vi "ATM Scaffold.vi"() -> ()   [LabVIEW 2026]
doc: "ATM controller for the CLD ATM exam, built on the Bank DQMH module. An event loop (producer) turns every front panel action into a command string on a queue - Insert Card, Terminate, Enter=<User Input>, the action of a pressed menu button, or Activity for a keystroke - so the value the consumer needs travels with the command. A command loop (consumer) dequeues them and runs the state machine in Handle ATM Command.vi, which asks the Bank module for every account operation; the GUI never touches the accounts file. Apply ATM UI State.vi then enables, disables, focuses and fills the panel for the new mode. A dequeue timeout of 10 s after card insertion is the inactivity timer, and every keystroke in User Input re-arms it. Return Card, the timeout and an error release Card Simulator with a signalling write, which ends the event loop and, through Terminate, the command loop. Shut Down ATM.vi then releases the queue, closes the panel reference and stops the Bank module."
panel:
  out "Right Menu":T1
  out "Left Menu":T1
  out "ATM Messages":string
  in  "Right Buttons":T2
  in  "Left Buttons":T2
  in  "User Input":string
  in  "Enter":bool
  in  "Card Simulator":bool
  out "error out":errorcluster
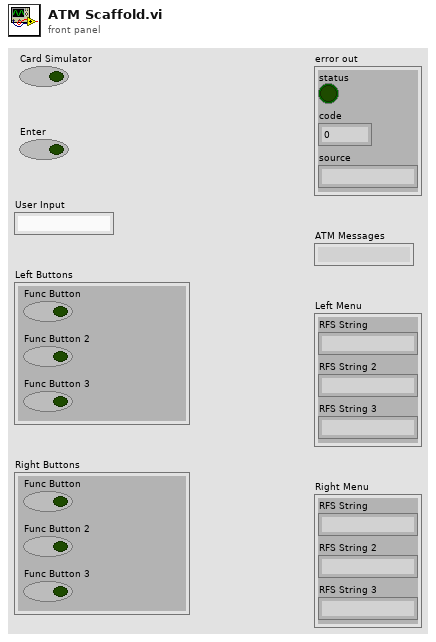
[diagram p1: front panel]
types:
  T1 = cluster{"RFS String":string, "RFS String 2":string, "RFS String 3":string}
  T2 = cluster{"Func Button":bool, "Func Button 2":bool, "Func Button 3":bool}
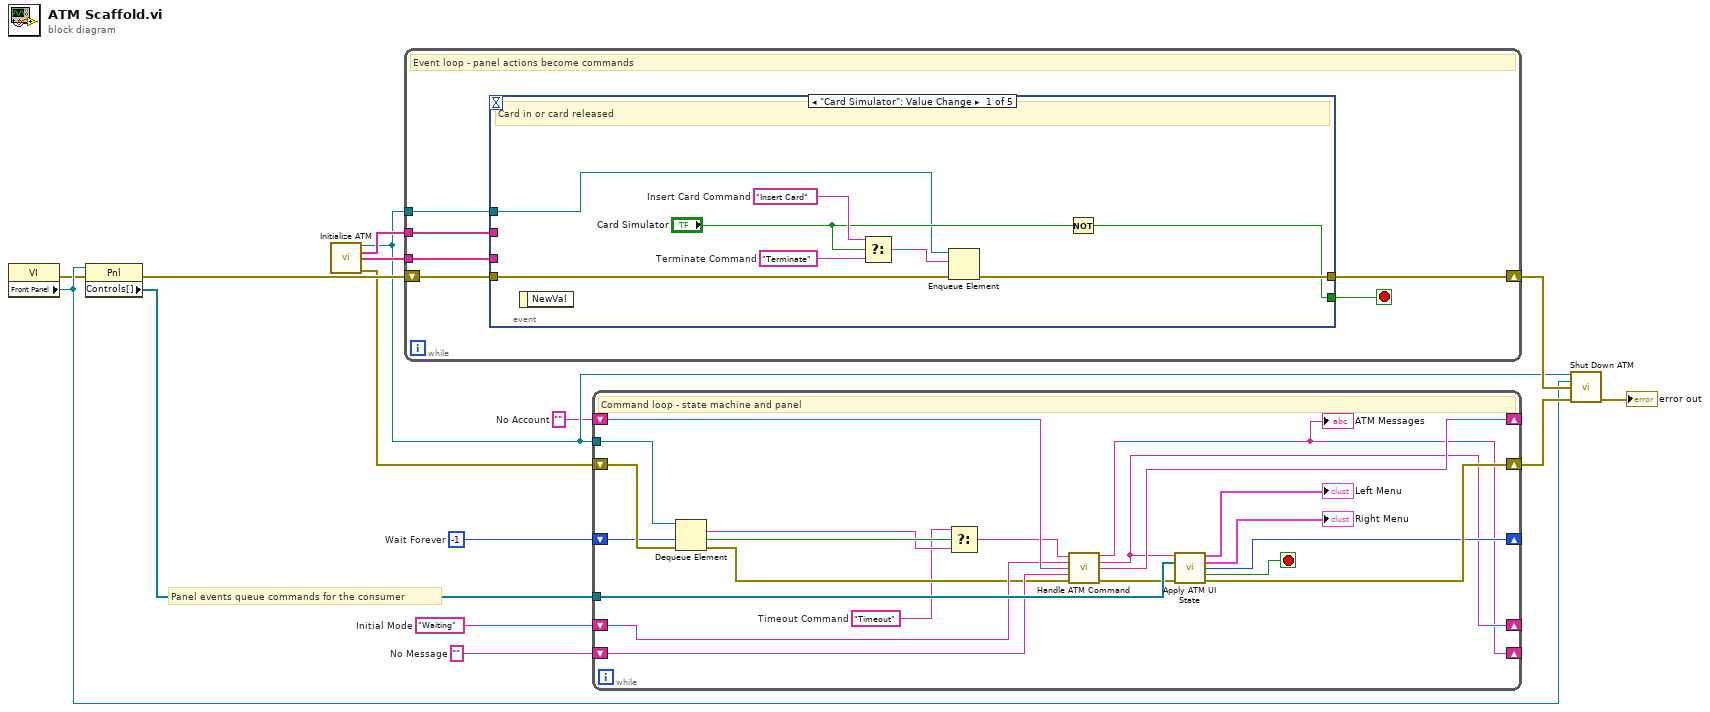
[diagram p0: block diagram]
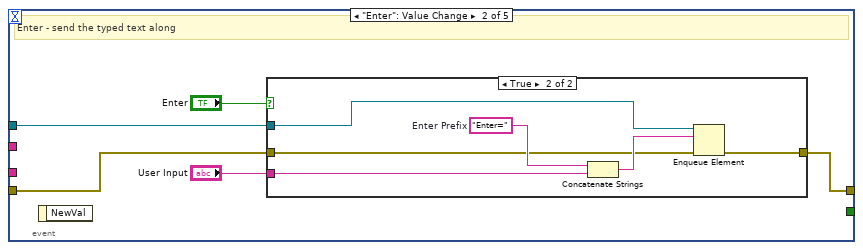
[diagram p2: hidden frame]
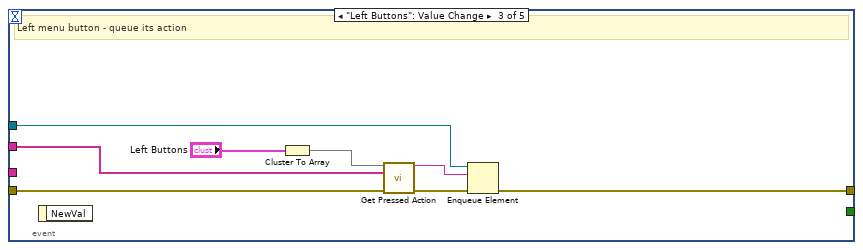
[diagram p4: hidden frame]
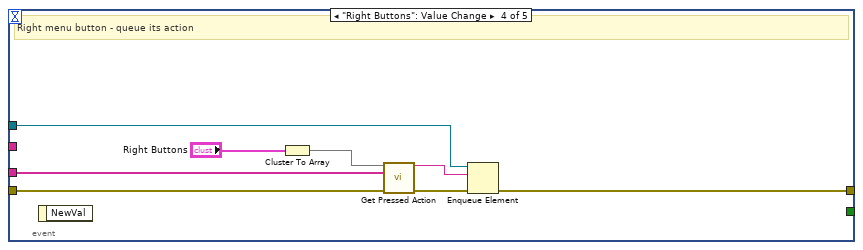
[diagram p5: hidden frame]
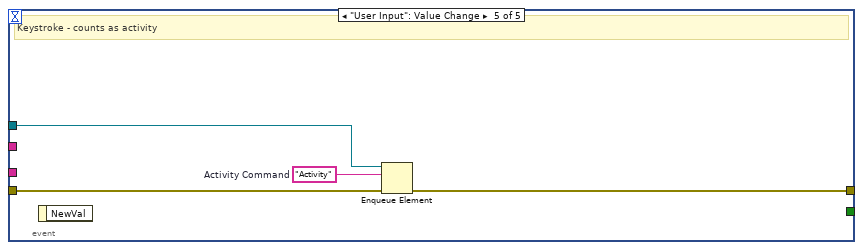
[diagram p6: hidden frame]
diagram:
  w4 = ""  # No Message
  w3 = ""  # No Account
  w2 = "Waiting"  # Initial Mode
  w1 = -1  # Wait Forever
  # "Panel events queue commands for the consumer"
  n1 = property class="VI"() -> (error out=w10:errorcluster, "Front Panel"=w11:refnum<vi>)  [unwired: 2 in, 1 out]
  n2 = property class="Pnl"(reference=w11, error in=w10) -> (error out=w12:errorcluster, "Controls[]"=w13:refnum<vi>[])  [unwired: 1 out]
  n3 = call "Initialize ATM.vi"() -> ("Command Queue"=w6:refnum<queue>, "Left Actions"=w7:string[], "Right Actions"=w8:string[], "error out"=w9:errorcluster)  [unwired: 12 in]
  n4 = while {
    tunnel: w6 -> [w16]
    tunnel: w7 -> [w17]
    tunnel: w8 -> [w18]
    shift-right: [w21] -> w14
    shift-left: w12 -> [w19]
    stop <- w20 stop-if-true
    # "Event loop - panel actions become commands"
    n5 = event shown="[0] \"Card Simulator\": Value Change" {
      selector: _ -> [_ _ _ _ _]
      dyn-events: _ -> [_ _ _ _ _]
      timeout: _ -> [_ _ _ _ _]
      tunnel: [w24 _ _ _ _] -> w20
      tunnel: w16 -> [w22 w30 w42 w50 w58]
      tunnel: w17 -> [_ _ w43 _ _]
      tunnel: w18 -> [_ _ _ w51 _]
      tunnel: w19 -> [w23 w31 w44 w52 w59]
      tunnel: [w25 w32 w45 w53 w60] -> w21
      event "Card Simulator": Value Change {
        w28 = "Terminate"  # Terminate Command
        w27 = "Insert Card"  # Insert Card Command
        # "Card in or card released"
        n6 = event-data() -> ()  [unwired: 1 in, 1 out]
        n7 = Select(t=w27, s="Card Simulator", f=w28) -> (s? t:f=w29:string)
        n8 = Enqueue Element(queue=w22, element=w29, error in (no error)=w23) -> (error out=w25:errorcluster)  [unwired: 1 in, 2 out]
        n9 = Not(x="Card Simulator") -> (.not. x?=w24:bool)
      }
      event "Enter": Value Change {
        # "Enter - send the typed text along"
        n10 = event-data() -> ()  [unwired: 1 in, 1 out]
        n11 = case shown="True" "Enter" {
          tunnel: "User Input" -> [_ w37]
          tunnel: w30 -> [_ w36]
          tunnel: w31 -> [w35 w38]
          tunnel: [w35 w39] -> w32
          frame False {
          }
          frame True {
            w40 = "Enter="  # Enter Prefix
            n12 = Concatenate Strings(w40, w37) -> (w41:string)
            n13 = Enqueue Element(queue=w36, element=w41, error in (no error)=w38) -> (error out=w39:errorcluster)  [unwired: 1 in, 2 out]
          }
        }
      }
      event "Left Buttons": Value Change {
        # "Left menu button - queue its action"
        n14 = event-data() -> ()  [unwired: 1 in, 1 out]
        n15 = Cluster To Array(cluster="Left Buttons") -> (array=w47:bool[])
        n16 = call "Get Pressed Action.vi"("Buttons"=w47, "Actions"=w43, "error in"=w44) -> ("Action"=w48:string, "error out"=w49:errorcluster)  [unwired: 11 in]
        n17 = Enqueue Element(queue=w42, element=w48, error in (no error)=w49) -> (error out=w45:errorcluster)  [unwired: 1 in, 2 out]
      }
      event "Right Buttons": Value Change {
        # "Right menu button - queue its action"
        n18 = event-data() -> ()  [unwired: 1 in, 1 out]
        n19 = Cluster To Array(cluster="Right Buttons") -> (array=w55:bool[])
        n20 = call "Get Pressed Action.vi"("Buttons"=w55, "Actions"=w51, "error in"=w52) -> ("Action"=w56:string, "error out"=w57:errorcluster)  [unwired: 11 in]
        n21 = Enqueue Element(queue=w50, element=w56, error in (no error)=w57) -> (error out=w53:errorcluster)  [unwired: 1 in, 2 out]
      }
      event "User Input": Value Change {
        w61 = "Activity"  # Activity Command
        # "Keystroke - counts as activity"
        n22 = event-data() -> ()  [unwired: 1 in, 1 out]
        n23 = Enqueue Element(queue=w58, element=w61, error in (no error)=w59) -> (error out=w60:errorcluster)  [unwired: 1 in, 2 out]
      }
    }
  }
  n24 = while {
    shift-right: [w73] -> _
    shift-left: w2 -> [w76]
    shift-right: [w74] -> _
    shift-left: w3 -> [w77]
    shift-right: [w63] -> _
    shift-left: w4 -> [w78]
    shift-right: [w79] -> _
    shift-left: w1 -> [w70]
    tunnel: w6 -> [w69]
    shift-right: [w81] -> w15
    shift-left: w9 -> [w71]
    tunnel: w13 -> [w82]
    stop <- w80 stop-if-true
    w62 = "Timeout"  # Timeout Command
    # "Command loop - state machine and panel"
    n25 = Dequeue Element(queue=w69, timeout in ms (-1)=w70, error in (no error)=w71) -> (element=w66:string, timed out?=w67:bool, error out=w68:errorcluster)  [unwired: 1 out]
    n26 = Select(t=w62, s=w67, f=w66) -> (s? t:f=w72:string)
    n27 = call "Handle ATM Command.vi"("Command"=w72, "Mode"=w76, "Account Number"=w77, "Current Message"=w78, "error in"=w68) -> ("Message"=w63:string, "New Mode"=w73:string, "Session Account"=w74:string, "error out"=w75:errorcluster)  [unwired: 7 in]
    "ATM Messages" <- w63
    n28 = call "Apply ATM UI State.vi"("Mode"=w73, "Panel Controls"=w82, "error in"=w75) -> ("Left Menu"=→"Left Menu":T1, "Right Menu"=→"Right Menu":T1, "Dequeue Timeout"=w79:i32, "Stop?"=w80:bool, "error out"=w81:errorcluster)  [unwired: 8 in]
  }
  n29 = call "Shut Down ATM.vi"("Command Queue"=w6, "Panel Reference"=w11, "Event Loop Error"=w14, "error in"=w15) -> ("error out"=→"error out":errorcluster)  [unwired: 11 in]
